vi "[ex ce]_Array - Building Arrays.vi"() -> ()   [LabVIEW 2021]
doc: "<B>Building arrays in a script</B>\n\nThe VI demonstrates a use of some functions to build 1D and 2D arrays.\n\n::: CalcExpress Toolkit :::\nCopyright (c) 2000-2026 Konstantin Shifershteyn. All rights reserved."
panel:
  out "ARR3":dbl[][](array[numeric])
  out "AR1":dbl[](array[numeric])
  in  "Expression":string="/* builds 1D array from scalars */\nAR1= vector(0,1,2);\n\n/* builds 1D array from scalars and 1D arrays */\nAR1= vector(AR1, AR1+3, 6,7 );\n\n/* builds 2D array from scalar & 1D array */\nARR2 = matrix( 111, vectorn(-1,5));\n\n/* builds 2D array from scalar, 1D array, and 2D array */\nARR3 = matrix(999, AR1, ARR2);"
  out "ARR2":dbl[][](array[numeric])
  # "resulting arrays"
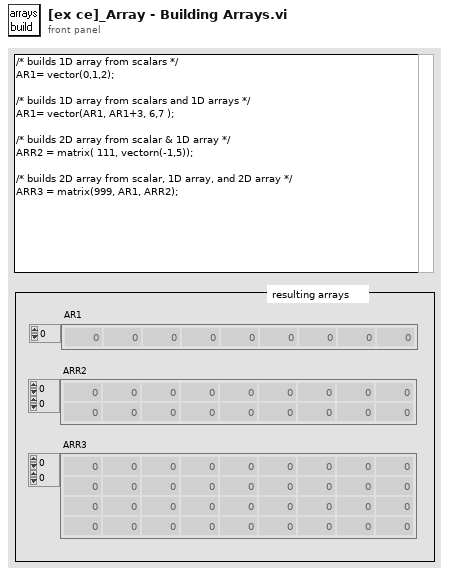
[diagram p1: front panel]
types:
  T1 = typedef "VarMan Variable Context Handle.ctl" = i32
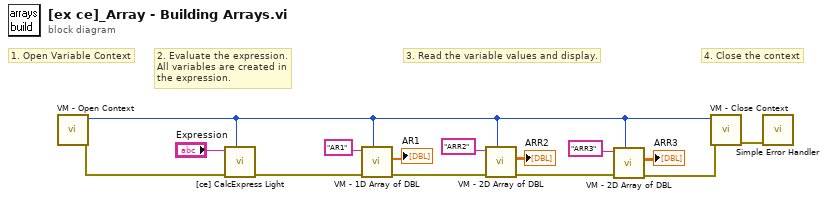
[diagram p0: block diagram]
diagram:
  # "4. Close the context"
  # "3. Read the variable values and display."
  # "2. Evaluate the expression.\nAll variables are created in\nthe expression."
  # "1. Open Variable Context"
  n1 = call "VM - Open Context.vi"() -> ("error out"=w9:errorcluster, "VC Handle out"=w1:T1)  [unwired: 9 in, 1 out]
  n2 = call "[ce] CalcExpress Light.vi"("VC Handle"=w1, "error in"=w9, "expression"="Expression") -> ("error out"=w7:errorcluster)  [unwired: 6 in, 2 out]
  n3 = call "VM - 1D Array of DBL.vi"("VC Handle"=w1, "error in"=w7, "name_spec"="AR1" ("name in")) -> ("error out"=w4:errorcluster, "value out"=→"AR1":dbl[])  [unwired: 3 in, 4 out]
  n4 = call "VM - 2D Array of DBL.vi"("VC Handle"=w1, "error in"=w4, "name_spec"="ARR2" ("name in")) -> ("error out"=w3:errorcluster, "value out"=→"ARR2":dbl[][])  [unwired: 3 in, 4 out]
  n5 = call "VM - 2D Array of DBL.vi"("VC Handle"=w1, "error in"=w3, "name_spec"="ARR3" ("name in")) -> ("error out"=w2:errorcluster, "value out"=→"ARR3":dbl[][])  [unwired: 3 in, 4 out]
  n6 = call "VM - Close Context.vi"("error in"=w2, "VC Handle"=w1) -> ("error out"=w8:errorcluster)  [unwired: 8 in, 1 out]
  n7 = call <vilib>:"Simple Error Handler.vi"("error in (no error)"=w8) -> ()  [unwired: 4 in, 5 out]
